vi "SLSC Get Plugin Path.vi"(9 "Type":string="_pinout.png", 10 "number":i32, 11 "Vendor Prefix":string) -> (3 "appended path":path)   [LabVIEW 2020, in "SLSC EDS System Explorer.lvlib"]
uses:
  SLSC EDS System Explorer.lvlib
  <vilib>/Utility/sysdir.llb/System Directory Type.ctl
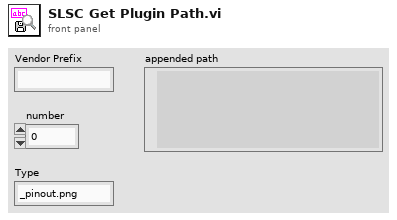
[diagram p1: front panel]
types:
  T1 = typedef "System Directory Type.ctl" = i32
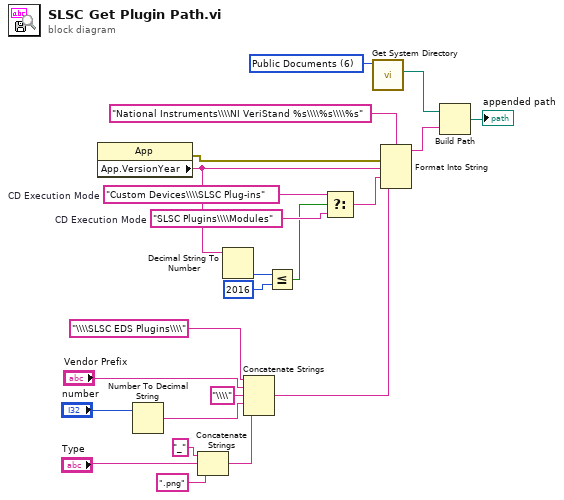
[diagram p0: block diagram]
diagram:
  w15 = "SLSC Plugins\\\\Modules"  # CD Execution Mode
  w16 = "Custom Devices\\\\SLSC Plug-ins"  # CD Execution Mode
  w7 = T1 6 items=["User Home"=0, "User Desktop"=1, "User Documents"=2, "User Application Data"=3, "User Preferences"=4, "User Temporary"=5, "Public Documents"=6, "Public Application Data"=7, "Public Preferences"=8, "Public Cache"=13, "System Core Libraries"=9, "System Installed Libraries"=10, "Application Files"=11, "Boot Volume Root"=12] ("system directory type")
  n1 = property class="App"() -> (error out=w8:errorcluster, "App.VersionYear"=w10:string)  [unwired: 2 in, 1 out]
  n2 = Number To Decimal String(number="number") -> (decimal integer string=w19:string)  [unwired: 1 in]
  n3 = Concatenate Strings("_" ("string"), "Type", ".png" ("string")) -> (w1:string)
  n4 = Decimal String To Number(string=w10) -> (number=w11:i32)  [unwired: 2 in, 1 out]
  n5 = Concatenate Strings("\\\\SLSC EDS Plugins\\\\" ("string"), "Vendor Prefix", "\\\\" ("string"), w19, w1) -> (w20:string)
  n6 = Less Or Equal?(x=w11, y=2016) -> (x <= y?=w14:bool)
  n7 = Select(t=w16, s=w14, f=w15) -> (s? t:f=w13:string)
  n8 = call <vilib>:"Get System Directory.vi"("system directory type"=w7) -> ("system directory"=w6:path)  [unwired: 10 in]
  n9 = Format Into String(format string="National Instruments\\\\NI VeriStand %s\\\\%s\\\\%s" ("name or relative path"), error in=w8, w10, w13, w20) -> (resulting string=w5:string)  [unwired: 1 in, 1 out]
  n10 = Build Path(base path=w6, name or relative path=w5) -> (appended path=→"appended path":path)
